vi "Evaluate Conditions.vi"(10 "Channel Feedback":T1, 11 "conditions":T3[](array[typedef])) -> (1 "measured":dbl, 2 "all found":bool=TRUE, 3 "all within":bool=TRUE, 4 "missing channel":string, 6 "target":dbl)   [LabVIEW 2026]
doc: "Evaluates a list of conditions against a Channel Feedback: all within is the AND of UE_Within_Tolerance per condition; all found is the AND of each channel being present; measured and target come from the first condition NOT within (else the last condition); missing channel is the first condition whose channel is absent. Empty conditions give all within TRUE and all found TRUE. Pure function, no error terminals, AF-free."
uses:
  Typedefs/Channel Feedback.ctl
  Typedefs/Channel Value.ctl
  Typedefs/Condition.ctl
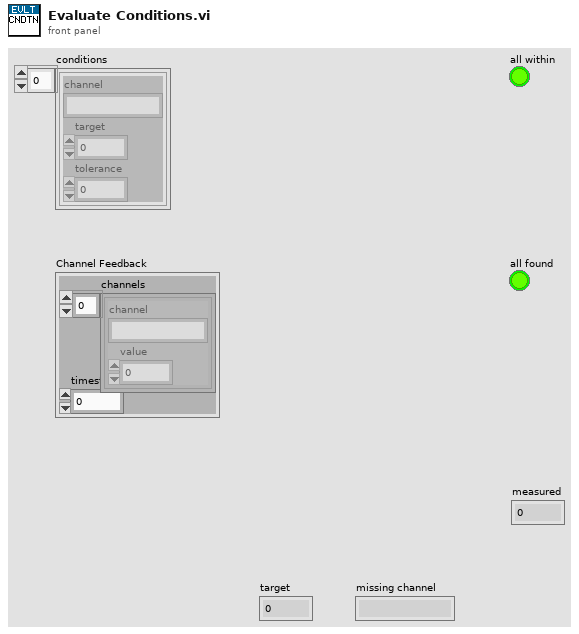
[diagram p1: front panel]
types:
  T1 = typedef "Channel Feedback.ctl" = cluster{"channels":T2[], "timestamp_ms":dbl}
  T2 = typedef "Channel Value.ctl" = cluster{"channel":string, "value":dbl}
  T3 = typedef "Condition.ctl" = cluster{"channel":string, "target":dbl, "tolerance":dbl}
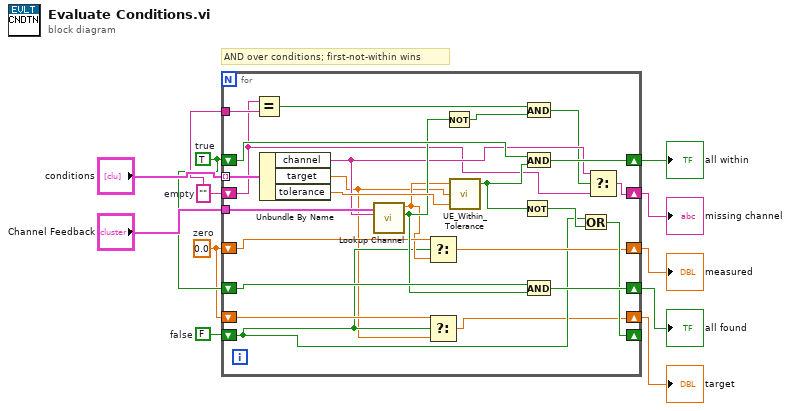
[diagram p0: block diagram]
diagram:
  w6 = ""  # empty
  w8 = 0.0  # zero
  w7 = FALSE  # false
  w9 = TRUE  # true
  # "AND over conditions; first-not-within wins"
  n1 = for {
    tunnel: "conditions" -> [w36] mode=indexing
    tunnel: "Channel Feedback" -> [w35]
    shift-right: [w32] -> w5
    shift-left: w9 -> [w33]
    shift-right: [w30] -> w4
    shift-left: w9 -> [w31]
    shift-right: [w16] -> w3
    shift-left: w8 -> [w18]
    shift-right: [w12] -> w2
    shift-left: w8 -> [w15]
    shift-right: [w19] -> w1
    shift-left: w6 -> [w20]
    shift-right: [w27] -> _
    shift-left: w7 -> [w14]
    tunnel: w6 -> [w25]
    n2 = Equal?(x=w20, y=w25) -> (x = y?=w24:bool)
    n3 = Unbundle By Name(w36) -> ("channel"=w22:string, "target"=w13:dbl, "tolerance"=w34:dbl)
    n4 = call "Lookup Channel.vi"("channel"=w22, "Channel Feedback"=w35) -> ("found"=w26:bool, "value"=w17:dbl)  [unwired: 8 in]
    n5 = Select(t=w18, s=w14, f=w17) -> (s? t:f=w16:dbl)
    n6 = Select(t=w15, s=w14, f=w13) -> (s? t:f=w12:dbl)
    n7 = Not(x=w26) -> (.not. x?=w23:bool)
    n8 = call "UE_Within_Tolerance.vi"("tolerance"=w34, "target"=w13, "actual"=w17) -> ("within_tolerance"=w29:bool)  [unwired: 2 in]
    n9 = Not(x=w29) -> (.not. x?=w28:bool)
    n10 = And(x=w24, y=w23) -> (x .and. y?=w21:bool)
    n11 = And(x=w33, y=w29) -> (x .and. y?=w32:bool)
    n12 = And(x=w31, y=w26) -> (x .and. y?=w30:bool)
    n13 = Or(x=w14, y=w28) -> (x .or. y?=w27:bool)
    n14 = Select(t=w22, s=w21, f=w20) -> (s? t:f=w19:string)
  }
  "all within" <- w5
  "all found" <- w4
  "measured" <- w3
  "target" <- w2
  "missing channel" <- w1
